vi "Two Way Event Recorder Initialization VI.vi"(8 "error in (no error)":errorcluster, 10 "Custom XML":string, 11 "Device Item Ref in":T1 format="%.0x") -> (0 "error out":errorcluster, 3 "Device Item Ref out":T1 format="%.0x")   [LabVIEW 2017, in "Two Way Event Recorder Custom Device.lvlib"]
uses:
  Two Way Event Recorder Custom Device.lvlib
  <vilib>/NI Veristand/Custom Device API/Custom Device Item Ref.ctl
  Simulator Inputs.ctl
  <vilib>/NI Veristand/Custom Device API/Custom Device Waveform.ctl
  <vilib>/NI Veristand/Custom Device API/Custom Device Waveform DataType.ctl
  Simulator Waveforms DBL.ctl
  Simulator Outputs.ctl
  <vilib>/NI Veristand/Custom Device API/Custom Device Channel.ctl
  <vilib>/NI Veristand/Custom Device API/Custom Device Channel Type.ctl
  <vilib>/NI Veristand/Custom Device API/Custom Device API.lvlib
  <vilib>/Utility/Data Type/NI_Data Type.lvlib
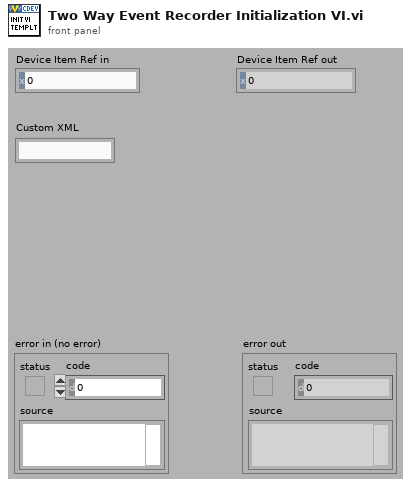
[diagram p1: front panel]
types:
  T1 = typedef "Custom Device API.lvlib/Custom Device Item Ref.ctl" = u64
  T2 = typedef "Custom Device API.lvlib/Custom Device Waveform.ctl" = cluster{"Data Type":T3, "Units":string}
  T3 = typedef "Custom Device API.lvlib/Custom Device Waveform DataType.ctl" = enum16{"Double", "Complex Double"}
  T4 = typedef "Custom Device API.lvlib/Custom Device Channel Type.ctl" = enum16{"Input", "Output"}
  T5 = typedef "Custom Device API.lvlib/Custom Device Channel.ctl" = cluster{"Type":T4, "Units":string, "Default Value":dbl, "Faultable":bool, "Scalable":bool}
  T6 = typedef "Two Way Event Recorder Custom Device.lvlib/Simulator Outputs.ctl" = enum16{"Baud Rate"}
  T7 = typedef "Simulator Waveforms DBL.ctl" = enum16{"Character Stream", "TimeStamps"}
  T8 = typedef "Two Way Event Recorder Custom Device.lvlib/Simulator Inputs.ctl" = enum16{"Enable Tx Msg", "Tx Msg Type", "Tx Msg Rate", "Tx Settings Visible"}
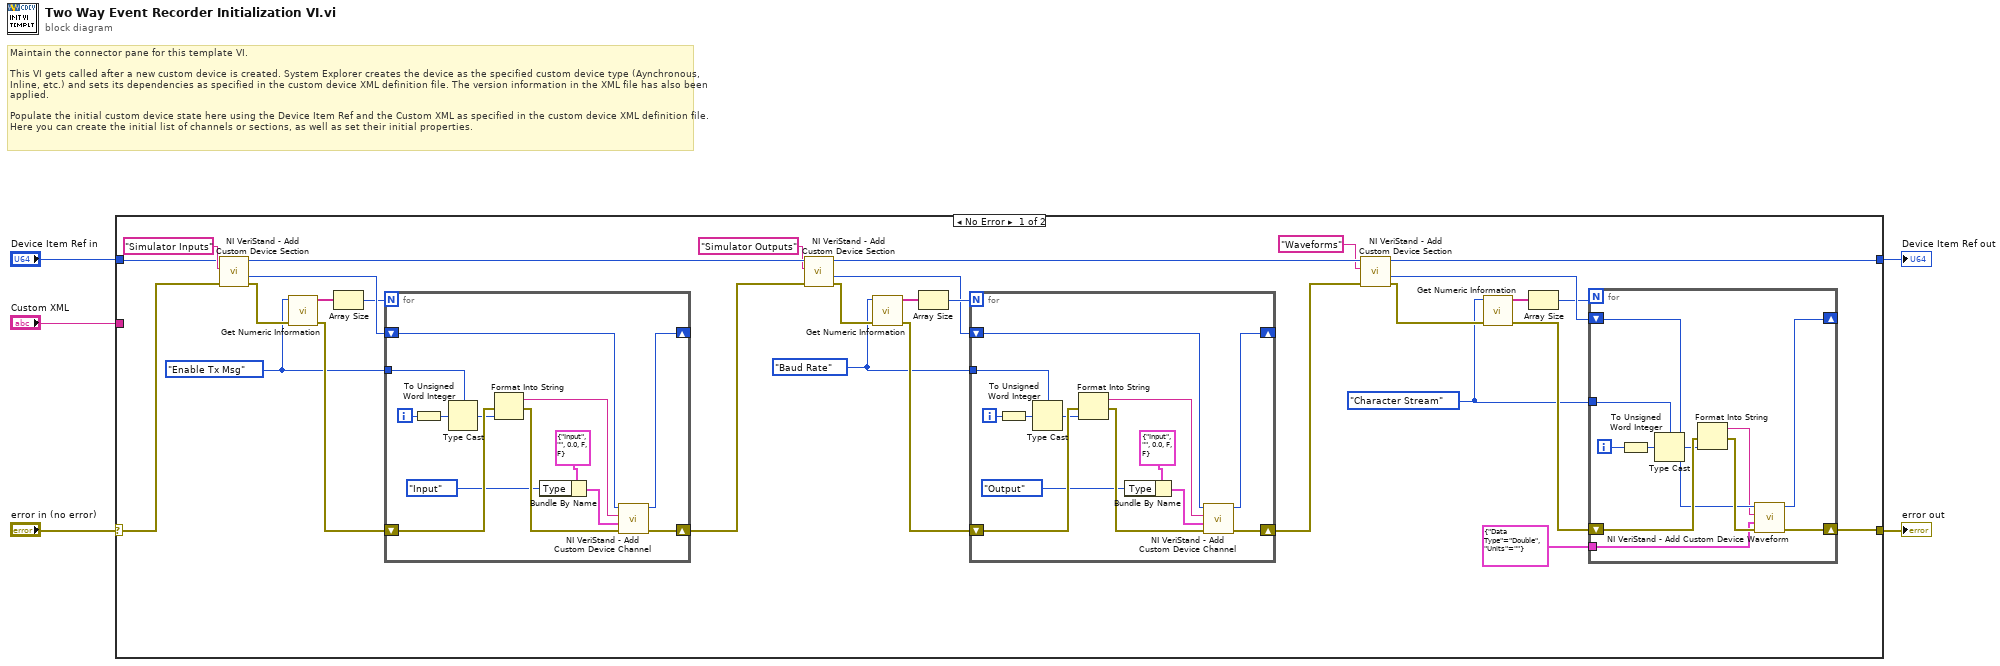
[diagram p0: block diagram]
diagram:
  # "Maintain the connector pane for this template VI.\n\nThis VI gets called after a new custom device is created. System Explorer creates the device as the specified custom device type (Aynchronous, Inline, etc.) and sets its dependencies as specified in the custom device XML definition file. The version information in the XML file has also been applied.\n\nPopulate the initial custom device state here using the Device Item Ref and the Custom XML as specified in the custom device XML definition file. Here you can create the initial list of channels or sections, as well as set their initial properties."
  n1 = case shown="No Error" "error in (no error)" {
    selector: "error in (no error)" -> [w25 w74]
    tunnel: [w18 w74] -> w5
    tunnel: [w21 w73] -> w3
    tunnel: "Device Item Ref in" -> [w24 w73]
    tunnel: "Custom XML" -> [_ _]
    frame No Error {
      w7 = Simulator_Outputs."Baud Rate" ("Inputs")
      w15 = Simulator_Waveforms_DBL."Character Stream" ("Waveforms")
      w23 = Simulator_Inputs."Enable Tx Msg" ("Inputs")
      n2 = call <vilib>:"NI VeriStand - Add Custom Device Section.vi"("error in (no error)"=w25, "Section Name"="Simulator Inputs", "Parent Ref in"=w24) -> ("error out"=w28:errorcluster, "Section Ptr"=w29:T1, "Parent Ref out"=w35:T1)  [unwired: 5 in, 1 out]
      n3 = call <vilib>:"Get Numeric Information.vi"("error in (no error)"=w28, "Variant"=w23) -> ("error out"=w27:errorcluster, "Enum Names"=w31:string[])  [unwired: 6 in, 2 out]
      n4 = Array Size(array=w31) -> (size(s)=w26:i32)
      n5 = for {
        N: w26 -> [_]
        shift-right: [w48] -> w8
        shift-left: w27 -> [w45]
        shift-right: [w46] -> _
        shift-left: w29 -> [w47]
        tunnel: w23 -> [w41]
        i -> [w37]
        n6 = To Unsigned Word Integer(number=w37) -> (unsigned 16bit integer=w36:u16)
        n7 = Type Cast(type=w41, x=w36) -> (*(type *) &x=w42:T8)
        n8 = Format Into String(error in=w45, w42) -> (resulting string=w43:string, error out=w44:errorcluster)  [unwired: 2 in]
        n9 = Bundle By Name(cluster=T5 {"Type"=enum."Input", "Units"="", "Default Value"=0.0, "Faultable"=FALSE, "Scalable"=FALSE} ("Channel"), "Type"=Custom_Device_Channel_Type."Input") -> (w39:T5)
        n10 = call <vilib>:"NI VeriStand - Add Custom Device Channel.vi"("error in (no error)"=w44, "Channel"=w39, "Channel Name"=w43, "Parent Ref in"=w47) -> ("error out"=w48:errorcluster, "Parent Ref out"=w46:T1)  [unwired: 4 in, 2 out]
      }
      n11 = call <vilib>:"NI VeriStand - Add Custom Device Section.vi"("error in (no error)"=w8, "Section Name"="Simulator Outputs", "Parent Ref in"=w35) -> ("error out"=w12:errorcluster, "Section Ptr"=w11:T1, "Parent Ref out"=w34:T1)  [unwired: 5 in, 1 out]
      n12 = call <vilib>:"Get Numeric Information.vi"("error in (no error)"=w12, "Variant"=w7) -> ("error out"=w13:errorcluster, "Enum Names"=w9:string[])  [unwired: 6 in, 2 out]
      n13 = Array Size(array=w9) -> (size(s)=w14:i32)
      n14 = for {
        N: w14 -> [_]
        shift-right: [w61] -> w6
        shift-left: w13 -> [w58]
        shift-right: [w59] -> _
        shift-left: w11 -> [w60]
        tunnel: w7 -> [w54]
        i -> [w50]
        n15 = To Unsigned Word Integer(number=w50) -> (unsigned 16bit integer=w49:u16)
        n16 = Type Cast(type=w54, x=w49) -> (*(type *) &x=w55:T6)
        n17 = Format Into String(error in=w58, w55) -> (resulting string=w56:string, error out=w57:errorcluster)  [unwired: 2 in]
        n18 = Bundle By Name(cluster=T5 {"Type"=enum."Input", "Units"="", "Default Value"=0.0, "Faultable"=FALSE, "Scalable"=FALSE} ("Channel"), "Type"=Custom_Device_Channel_Type."Output") -> (w52:T5)
        n19 = call <vilib>:"NI VeriStand - Add Custom Device Channel.vi"("error in (no error)"=w57, "Channel"=w52, "Channel Name"=w56, "Parent Ref in"=w60) -> ("error out"=w61:errorcluster, "Parent Ref out"=w59:T1)  [unwired: 4 in, 2 out]
      }
      n20 = call <vilib>:"NI VeriStand - Add Custom Device Section.vi"("error in (no error)"=w6, "Section Name"="Waveforms", "Parent Ref in"=w34) -> ("error out"=w32:errorcluster, "Section Ptr"=w20:T1, "Parent Ref out"=w21:T1)  [unwired: 5 in, 1 out]
      n21 = call <vilib>:"Get Numeric Information.vi"("error in (no error)"=w32, "Variant"=w15) -> ("error out"=w33:errorcluster, "Enum Names"=w17:string[])  [unwired: 6 in, 2 out]
      n22 = Array Size(array=w17) -> (size(s)=w16:i32)
      n23 = for {
        N: w16 -> [_]
        tunnel: T2 {"Data Type"=enum."Double", "Units"=""} ("Waveform") -> [w69]
        shift-right: [w68] -> w18
        shift-left: w33 -> [w72]
        tunnel: w15 -> [w66]
        shift-right: [w62] -> _
        shift-left: w20 -> [w70]
        i -> [w65]
        n24 = To Unsigned Word Integer(number=w65) -> (unsigned 16bit integer=w67:u16)
        n25 = Type Cast(type=w66, x=w67) -> (*(type *) &x=w64:T7)
        n26 = Format Into String(error in=w72, w64) -> (resulting string=w63:string, error out=w71:errorcluster)  [unwired: 2 in]
        n27 = call <vilib>:"NI VeriStand - Add Custom Device Waveform.vi"("error in (no error)"=w71, "Waveform"=w69, "Waveform Name"=w63, "Parent Ref in"=w70) -> ("error out"=w68:errorcluster, "Parent Ref out"=w62:T1)  [unwired: 4 in, 2 out]
      }
    }
    frame Error {
    }
  }
  "error out" <- w5
  "Device Item Ref out" <- w3
